vi "LVA_State.vi"(4 "SetDC":bool, 8 "error in (no error)":errorcluster, 10 "Get open VIs Argument":T3, 11 "Data Cluster 2":T1) -> (0 "error out":errorcluster, 3 "Data Cluster":T1)   [LabVIEW 2020, in "Scripting Server.lvlib"]
uses:
  Scripting Server.lvlib
  Get open VIs (Reply Payload)--cluster.ctl
  Get open VIs Argument--cluster.ctl
  Config Data.ctl
  Module Data--cluster.ctl
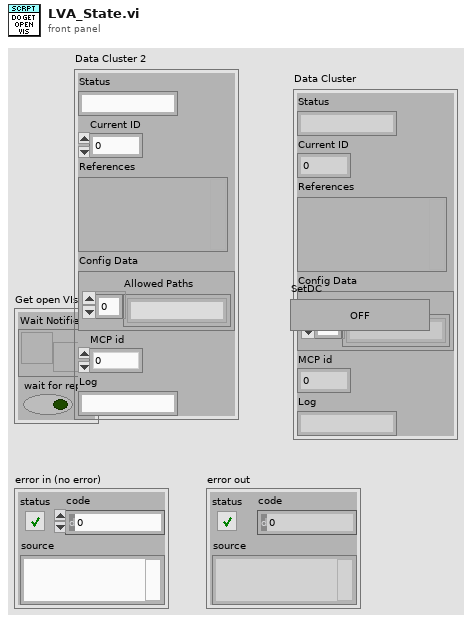
[diagram p1: front panel]
types:
  T1 = typedef "Scripting Server.lvlib/Module Data--cluster.ctl" = cluster{"Status":string, "Current ID":i32, "References":variant, "Config Data":T2, "MCP id":i32, "Log":string}
  T2 = typedef "Scripting Server.lvlib/Config Data.ctl" = cluster{"Allowed Paths":string[]}
  T3 = typedef "Scripting Server.lvlib/Get open VIs Argument--cluster.ctl" = cluster{"Wait Notifier":refnum<notifier>, "wait for reply":bool}
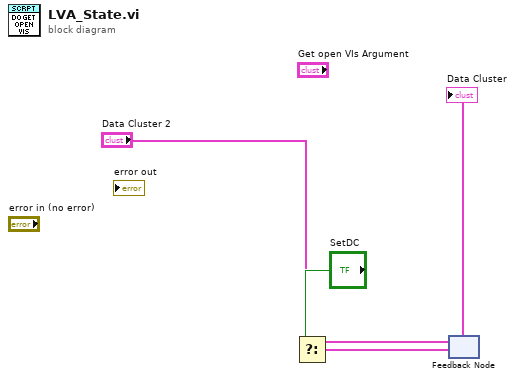
[diagram p0: block diagram]
diagram:
  n1 = feedback #1 ("FN")() -> (w1:T1)  [unwired: 1 in]
  "Data Cluster" <- w1
  n2 = Select ("Sel")(t="Data Cluster 2", s="SetDC", f=w1) -> (s? t:f=w3:T1)
  n3 = feedback-in #1(w3) -> ()
